vi "VHistFile - Search time stamps subset.vi"(6 "time stamps":dbl[](array[numeric]) format="%<%H:%M:%S%2u\n%d/%m/%Y>T", 9 "time range":cluster{"t1":dbl, "t2":dbl} {"t2" format="%<%H:%M:%S%2u\n%d/%m/%Y>T"; "t1" format="%<%H:%M:%S%2u\n%d/%m/%Y>T"}) -> (2 "length":i32, 3 "index":i32)   [LabVIEW 2021]
doc: "::: CalcExpress Toolkit :::\nCopyright (c) 2000-2026 Konstantin Shifershteyn. All rights reserved."
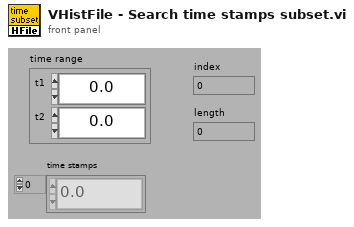
[diagram p1: front panel]
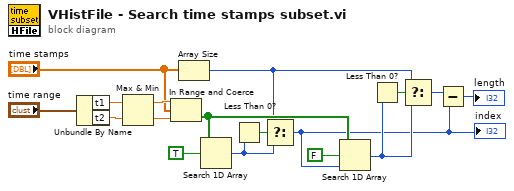
[diagram p0: block diagram]
diagram:
  n1 = Unbundle By Name("time range") -> ("t1"=w17:dbl, "t2"=w16:dbl)
  n2 = Max & Min(x=w17, y=w16) -> (max(x,y)=w13:dbl, min(x,y)=w12:dbl)
  n3 = In Range and Coerce(upper limit=w13, x="time stamps", lower limit=w12) -> (In Range?=w7:bool[])  [unwired: 1 out]
  n4 = Array Size(array="time stamps") -> (size(s)=w4:i32)
  n5 = Search 1D Array(1D array=w7, element=TRUE) -> (index of element=w2:i32)  [unwired: 1 in]
  n6 = Less Than 0?(x=w2) -> (x < 0?=w9:bool)
  n7 = Select(t=w4, s=w9, f=w2) -> (s? t:f=w1:i32)
  "index" <- w1
  n8 = Search 1D Array(1D array=w7, element=FALSE, start index (0)=w1) -> (index of element=w5:i32)
  n9 = Less Than 0?(x=w5) -> (x < 0?=w6:bool)
  n10 = Select(t=w4, s=w6, f=w5) -> (s? t:f=w3:i32)
  n11 = Subtract(x=w3, y=w1) -> (x-y=→"length":i32)
